vi "Const_ADO.vi"() -> (0 "ADOMapper":refnum<class "ADOMapper.lvclass">)   [LabVIEW 2026, in "ORM_ADONetCore.lvlib"]
uses:
  ORM_ADONetCore.lvlib
  ADOMapper/ADOMapper.lvclass
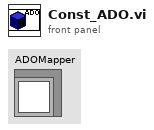
[diagram p1: front panel]
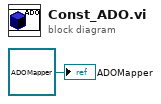
[diagram p0: block diagram]
diagram:
  "ADOMapper" <- refnum<class "ADOMapper.lvclass"> refnum ("ADONet.lvlib:ADOMapper.lvclass")
